vi "JSONRPC-InvokeMethod.vi"(7 "method":T1(ring), 8 "error in (no error)":errorcluster, 11 "params":string[](array[string])) -> (0 "error out":errorcluster, 3 "result":string)   [LabVIEW 2015]
doc: "Invokes the actual implementation of a RIP <b>method</b>."
uses:
  Configuration/Global_Configurations.vi
  JSONRPC-GetAsString.vi
  JSONRPC-ArrayToString_Cluster.vi
  JSONRPC-ArrayToString_String.vi
  JSONRPC-GetAsArray.vi
panel:
  # "InvokeMethod"
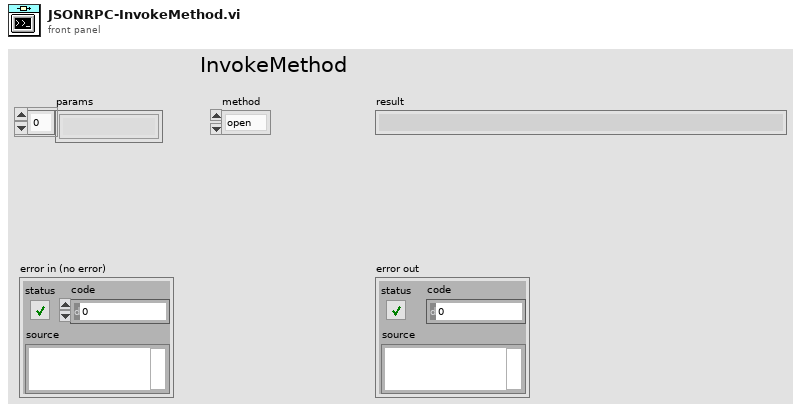
[diagram p1: front panel]
types:
  T1 = enum16{"open", "close", "start", "stop", "get", "set", "info", "UNDEFINED"}
  T2 = enum16{"Parse error", "Invalid request", "Method not found", "Invalid params", "Internal error", "Server error", ""}
  T3 = cluster{"Path":path, "Name":string, "Authors":string, "Keywords":string, "Description":string, "Cameras":cluster{"Base URL":string, "Path":string, "Name":string}[], "Sampling":cluster{"Sampled Variable":string, "Delta":dbl}[], "Sampling Freq":u32}[]
  T4 = cluster{"Name":string, "Type":string, "Min":string, "Max":string, "Precision":string, "Description":string}[]
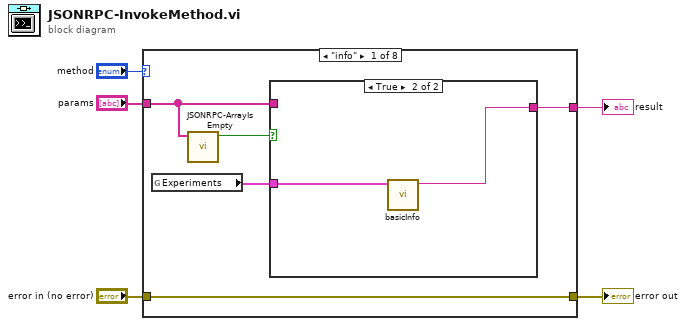
[diagram p0: block diagram]
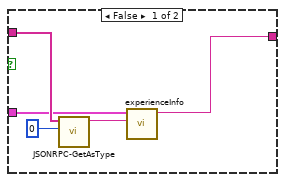
[diagram p2: hidden frame]
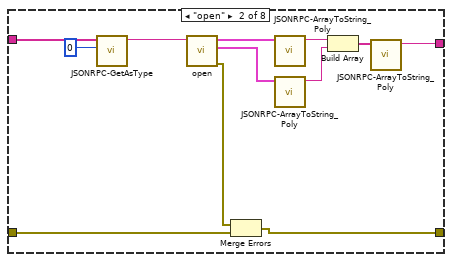
[diagram p3: hidden frame]
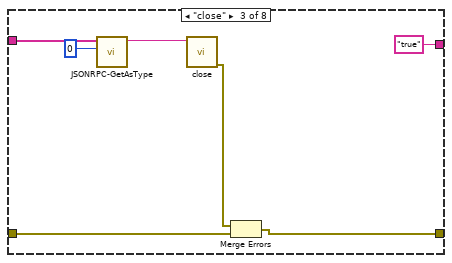
[diagram p4: hidden frame]
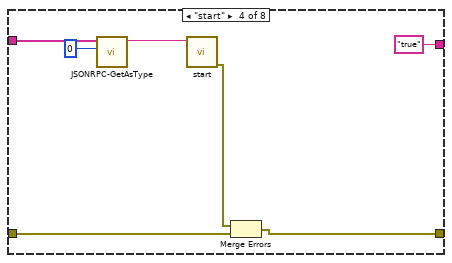
[diagram p5: hidden frame]
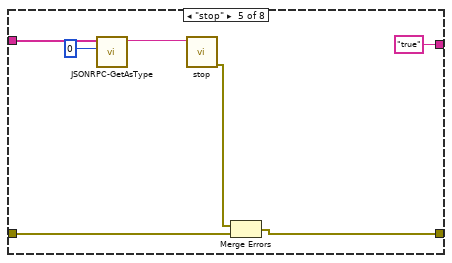
[diagram p6: hidden frame]
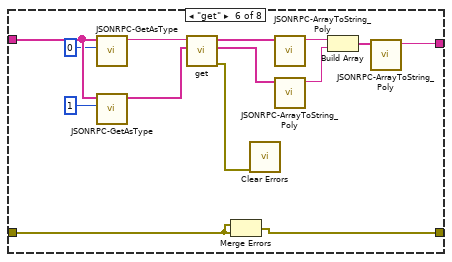
[diagram p7: hidden frame]
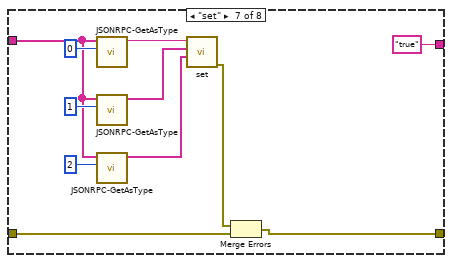
[diagram p8: hidden frame]
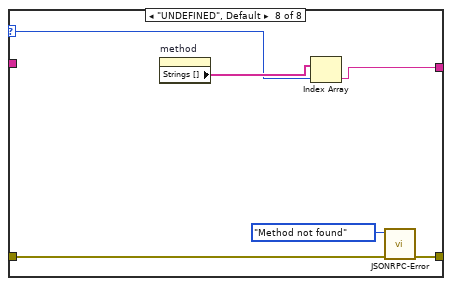
[diagram p9: hidden frame]
diagram:
  n1 = case shown="\"info\"" "method" {
    selector: "method" -> [_ _ _ _ _ _ _ w77]
    tunnel: "params" -> [w9 w22 w31 w38 w47 w58 w67 _]
    tunnel: [w10 w28 w34 w41 w48 w64 w73 w80] -> w3
    tunnel: "error in (no error)" -> [w10 w29 w35 w42 w49 w53 w74 w79]
    tunnel: [w7 w18 "true" "true" "true" w51 "true" w76] -> w1
    frame "info" {
      n2 = global read "Global_Configurations.vi" "Experiments"() -> (w6:T3)
      n3 = call "JSONRPC-ArrayIsEmpty.vi"("input array"=w9) -> ("empty?"=w8:bool)  [unwired: 10 in]
      n4 = case shown="True" w8 {
        tunnel: w9 -> [w12 _]
        tunnel: [w15 w17] -> w7
        tunnel: w6 -> [w11 w16]
        frame False {
          n5 = call-poly "JSONRPC-GetAsType.vi"("index"=0, "params"=w12) -> ("output"=w13:string)  [unwired: 9 in]
          n6 = call "experienceInfo.vi"("info in"=w13, "Experiments"=w11) -> ("info out"=w15:string)  [unwired: 9 in]
        }
        frame True {
          n7 = call "basicInfo.vi"("Experiments"=w16) -> ("String"=w17:string)  [unwired: 10 in]
        }
      }
    }
    frame "open" {
      n8 = call-poly "JSONRPC-GetAsType.vi"("index"=0, "params"=w22) -> ("output"=w23:string)  [unwired: 9 in]
      n9 = call "open.vi"("Experience ID"=w23) -> ("error out"=w27:errorcluster, "Indicators_list"=w19:T4, "Controls_list"=w20:T4)  [unwired: 8 in]
      n10 = Merge Errors(w27, w29) -> (w28:errorcluster)
      n11 = call-poly "JSONRPC-ArrayToString_Poly.vi"("List"=w20) -> ("Output"=w21:string)  [unwired: 10 in]
      n12 = call-poly "JSONRPC-ArrayToString_Poly.vi"("List"=w19) -> ("Output"=w26:string)  [unwired: 10 in]
      n13 = Build Array(w21, w26) -> (w25:string[])
      n14 = call-poly "JSONRPC-ArrayToString_Poly.vi"("Array"=w25) -> ("Output"=w18:string)  [unwired: 10 in]
    }
    frame "close" {
      n15 = call-poly "JSONRPC-GetAsType.vi"("index"=0, "params"=w31) -> ("output"=w32:string)  [unwired: 9 in]
      n16 = call "close.vi"("Experience ID"=w32) -> ("error out"=w36:errorcluster)  [unwired: 10 in]
      n17 = Merge Errors(w36, w35) -> (w34:errorcluster)
    }
    frame "start" {
      n18 = call-poly "JSONRPC-GetAsType.vi"("index"=0, "params"=w38) -> ("output"=w39:string)  [unwired: 9 in]
      n19 = call "start.vi"("Experience ID"=w39) -> ("error out"=w43:errorcluster)  [unwired: 10 in]
      n20 = Merge Errors(w43, w42) -> (w41:errorcluster)
    }
    frame "stop" {
      n21 = call-poly "JSONRPC-GetAsType.vi"("index"=0, "params"=w47) -> ("output"=w45:string)  [unwired: 9 in]
      n22 = call "stop.vi"("Experience ID"=w45) -> ("error out"=w50:errorcluster)  [unwired: 10 in]
      n23 = Merge Errors(w50, w49) -> (w48:errorcluster)
    }
    frame "get" {
      n24 = call-poly "JSONRPC-GetAsType.vi"("index"=0, "params"=w58) -> ("output"=w54:string)  [unwired: 9 in]
      n25 = call-poly "JSONRPC-GetAsType.vi"("index"=1, "params"=w58) -> ("output"=w55:string[])  [unwired: 9 in]
      n26 = call "get.vi"("variables"=w55, "Experience ID"=w54) -> ("error out"=w52:errorcluster, "values"=w62:string[], "names"=w60:string[])  [unwired: 7 in]
      n27 = Merge Errors(w53, w53) -> (w64:errorcluster)
      n28 = call <vilib>:"Clear Errors.vi"("error in (no error)"=w52) -> ()  [unwired: 5 in, 2 out]
      n29 = call-poly "JSONRPC-ArrayToString_Poly.vi"("Array"=w60) -> ("Output"=w59:string)  [unwired: 10 in]
      n30 = call-poly "JSONRPC-ArrayToString_Poly.vi"("Array"=w62) -> ("Output"=w63:string)  [unwired: 10 in]
      n31 = Build Array(w59, w63) -> (w61:string[])
      n32 = call-poly "JSONRPC-ArrayToString_Poly.vi"("Array"=w61) -> ("Output"=w51:string)  [unwired: 10 in]
    }
    frame "set" {
      n33 = call-poly "JSONRPC-GetAsType.vi"("index"=0, "params"=w67) -> ("output"=w72:string)  [unwired: 9 in]
      n34 = call-poly "JSONRPC-GetAsType.vi"("index"=1, "params"=w67) -> ("output"=w70:string[])  [unwired: 9 in]
      n35 = call-poly "JSONRPC-GetAsType.vi"("index"=2, "params"=w67) -> ("output"=w66:string[])  [unwired: 9 in]
      n36 = call "set.vi"("values"=w66, "variables"=w70, "Experience ID"=w72) -> ("error out"=w75:errorcluster)  [unwired: 8 in]
      n37 = Merge Errors(w75, w74) -> (w73:errorcluster)
    }
    frame "UNDEFINED", Default {
      n38 = property on="method" class="Enum (strict)"() -> ("Strings []"=w78:string[])  [unwired: 2 in, 2 out]
      n39 = Index Array(array=w78, index=w77) -> (element=w76:string)
      n40 = call "JSONRPC-Error.vi"("error in"=w79, "Type"=T2."Method not found") -> ("error out"=w80:errorcluster)  [unwired: 9 in]
    }
  }
  "error out" <- w3
  "result" <- w1
